vi "Ft to Encoder Velocity.vi"(11 "ft/s":dbl=30.0) -> (3 "v":dbl)   [LabVIEW 2023]
panel:
  in  "Wheel Radius (ft)":dbl=0.5 format="%#_13g"
  in  "Gear Ratio":dbl=8.46 format="%#_13g"
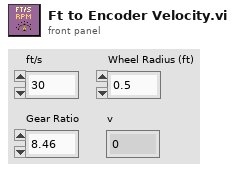
[diagram p1: front panel]
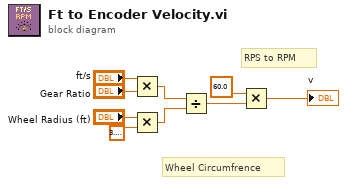
[diagram p0: block diagram]
diagram:
  # "RPS to RPM"
  # "Wheel Circumfrence"
  n1 = Multiply(x="ft/s", y="Gear Ratio") -> (x*y=w7:dbl)
  n2 = Multiply(x="Wheel Radius (ft)", y=3.141592653589793) -> (x*y=w4:dbl)
  n3 = Divide(x=w7, y=w4) -> (x/y=w2:dbl)
  n4 = Multiply(x=60.0, y=w2) -> (x*y=→"v":dbl)
